vi "Initialize Front Panel.vi"(8 "error in":errorcluster, 11 "Peer Review in":refnum<class "Peer Review.lvclass">) -> (0 "error out":errorcluster, 2 "Event Registration Refnum":refnum<event-registration>, 3 "Peer Review out":refnum<class "Peer Review.lvclass">)   [LabVIEW 2020, in "Peer Review.lvclass"]
uses:
  Peer Review.lvclass
  Peer Review.lvclass/Peer Review.ctl
  <vilib>/Utility/miscctls.llb/LVRowAndColumnTypeDef.ctl
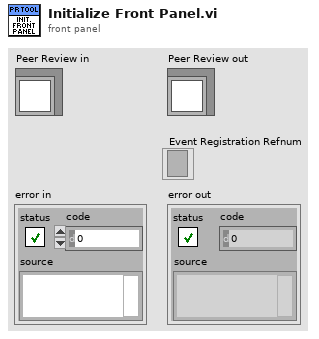
[diagram p1: front panel]
types:
  T1 = typedef "LVRowAndColumnTypeDef.ctl" = cluster{"Row":i32, "Column":i32}
  T2 = enum8{"Enabled", "Disabled", "Disabled and Grayed Out"}
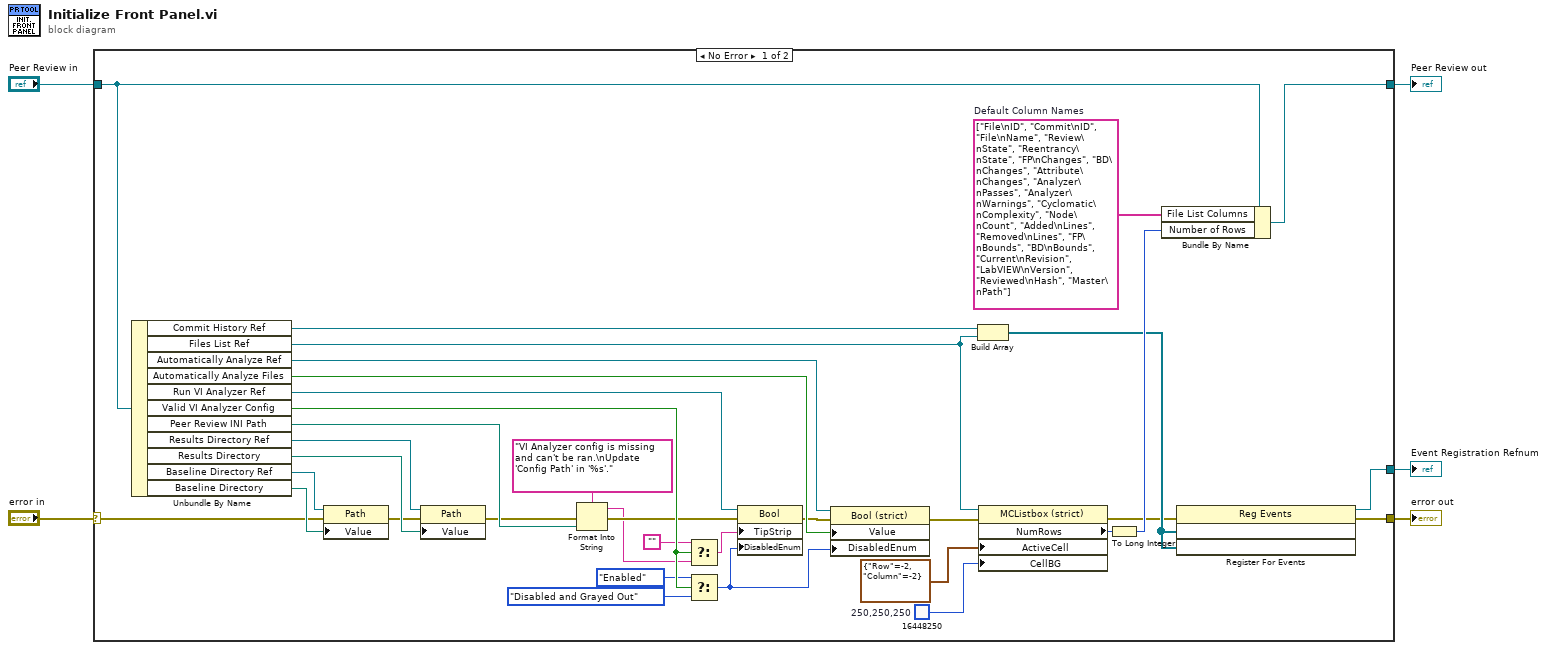
[diagram p0: block diagram]
diagram:
  n1 = case shown="No Error" "error in" {
    selector: "error in" -> [w33 w42]
    tunnel: [w19 w42] -> w4
    tunnel: [w17 w41] -> w2
    tunnel: "Peer Review in" -> [w16 w41]
    tunnel: [w18 _] -> w1
    frame No Error {
      w6 = u32 16448250  # 250,250,250
      w8 = string[] ["File\nID", "Commit\nID", "File\nName", "Review\nState", "Reentrancy\nState", "FP\nChanges", "BD\nChanges", "Attribute\nChanges", "Analyzer\nPasses", "Analyzer\nWarnings", "Cyclomatic\nComplexity", "Node\nCount", "Added\nLines", "Removed\nLines", "FP\nBounds", "BD\nBounds", "Current\nRevision", "LabVIEW\nVersion", "Reviewed\nHash", "Master\nPath"]  # Default Column Names
      n2 = Unbundle By Name(w16) -> ("Commit History Ref"=w20:refnum<vi>, "Files List Ref"=w9:refnum<vi>, "Automatically Analyze Ref"=w14:refnum<vi>, "Automatically Analyze Files"=w35:bool, "Run VI Analyzer Ref"=w30:refnum<vi>, "Valid VI Analyzer Config"=w40:bool, "Peer Review INI Path"=w37:path, "Results Directory Ref"=w31:refnum<vi>, "Results Directory"=w38:path, "Baseline Directory Ref"=w32:refnum<vi>, "Baseline Directory"=w39:path)
      n3 = property on="Property Node" class="Path"(reference=w32, error in=w33, "Value"=w39) -> (error out=w34:errorcluster)  [unwired: 1 out]
      n4 = property on="Property Node" class="Path"(reference=w31, error in=w34, "Value"=w38) -> (error out=w27:errorcluster)  [unwired: 1 out]
      n5 = Format Into String(format string="VI Analyzer config is missing and can't be ran.\nUpdate 'Config Path' in '%s'." ("f"), error in=w27, w37) -> (resulting string=w22:string, error out=w26:errorcluster)  [unwired: 1 in]
      n6 = Select(t="", s=w40, f=w22) -> (s? t:f=w21:string)
      n7 = Select(t=T2."Enabled" ("Disabled"), s=w40, f=T2."Disabled and Grayed Out" ("Disabled")) -> (s? t:f=w13:T2)
      n8 = property on="Property Node" class="Bool"(reference=w30, error in=w26, "TipStrip"=w21, "DisabledEnum"=w13) -> (error out=w15:errorcluster)  [unwired: 1 out]
      n9 = property on="Property Node" class="Bool (strict)"(reference=w14, error in=w15, "Value"=w35, "DisabledEnum"=w13) -> (error out=w11:errorcluster)  [unwired: 1 out]
      n10 = Build Array(w20, w9) -> (w24:refnum<vi>[])
      n11 = property class="MCListbox (strict)"(reference=w9, error in=w11, "ActiveCell"=T1 {"Row"=-2, "Column"=-2} ("Active Cell:Active Cell"), "CellBG"=w6) -> (error out=w10:errorcluster, "NumRows"=w12:u32)  [unwired: 1 out]
      n12 = To Long Integer(number=w12) -> (32bit integer=w36:i32)
      n13 = Bundle By Name(cluster=w16, "File List Columns"=w8, "Number of Rows"=w36) -> (w17:refnum<class "Peer Review.lvclass">)
      n14 = register-events(error in=w10, w24, w24) -> (reference out=w18:refnum<event-registration>, error out=w19:errorcluster)  [unwired: 1 in]
    }
    frame Error {
    }
  }
  "error out" <- w4
  "Peer Review out" <- w2
  "Event Registration Refnum" <- w1
